vi "Check Action.vi"(6 "HRS Time":dbl, 7 "Values In":dbl[](array[numeric]), 8 "error in (no error)":errorcluster, 11 "SequencedValves in":refnum<class "TriggerDelayControl.lvclass">) -> (0 "error out":errorcluster, 2 "Actions":T1[](array[typedef]), 3 "SequencedValves out":refnum<class "TriggerDelayControl.lvclass">, 5 "Values":dbl[](array[numeric]))   [LabVIEW 2020, in "VolatusControl.lvlib" / "TriggerDelayControl.lvclass"]
uses:
  TriggerDelayControl.lvclass
  Control Action.ctl
  TriggerDelayControl.lvclass/TriggerDelayControl.ctl
  State.ctl
  Volatus/MessageQ/MessageQ.lvclass
  VolatusControl.lvlib
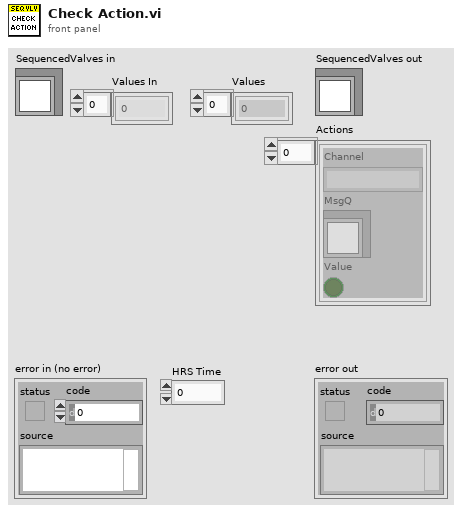
[diagram p1: front panel]
types:
  T1 = typedef "VolatusControl.lvlib/Control Action.ctl" = cluster{"Channel":string, "MsgQ":refnum<class "MessageQ.lvclass">, "Value":bool}
  T2 = typedef "VolatusControl.lvlib/TriggerDelayControl.lvclass/State.ctl" = enum16{"Idle", "Start", "Check", "Delay", "Triggered"}
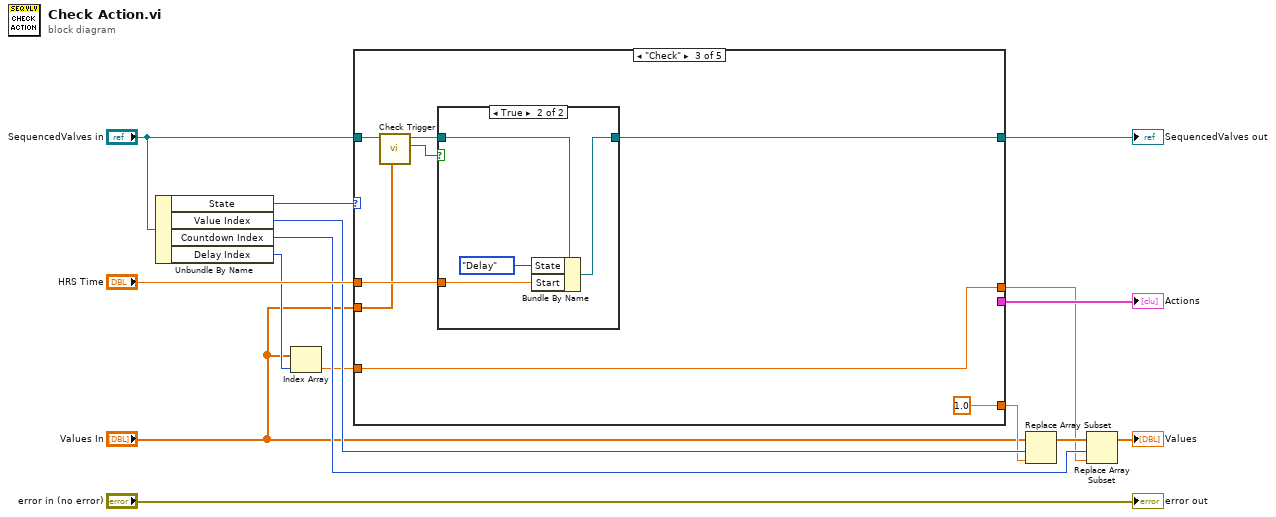
[diagram p0: block diagram]
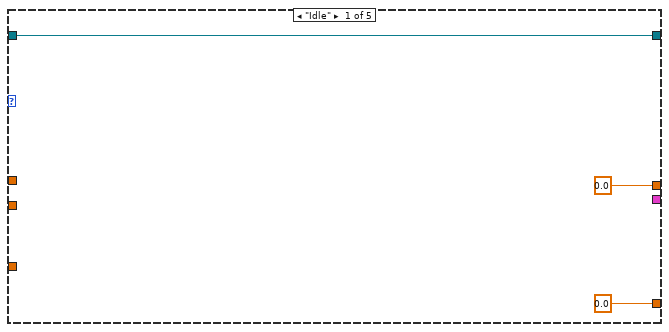
[diagram p2: hidden frame]
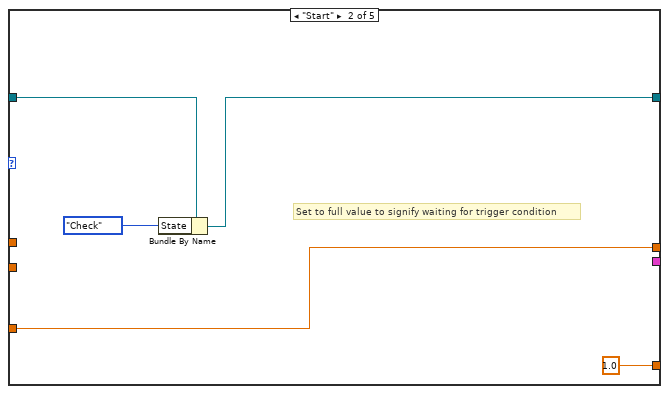
[diagram p3: hidden frame]
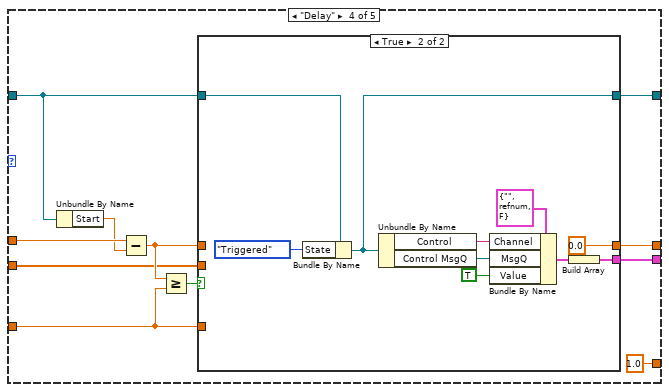
[diagram p5: hidden frame]
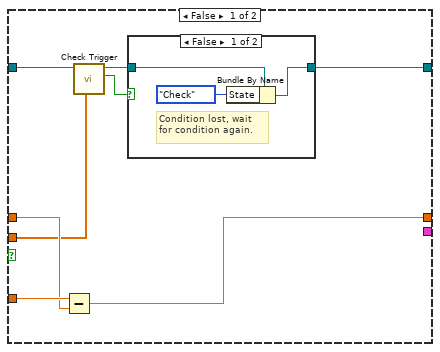
[diagram p6: hidden frame]
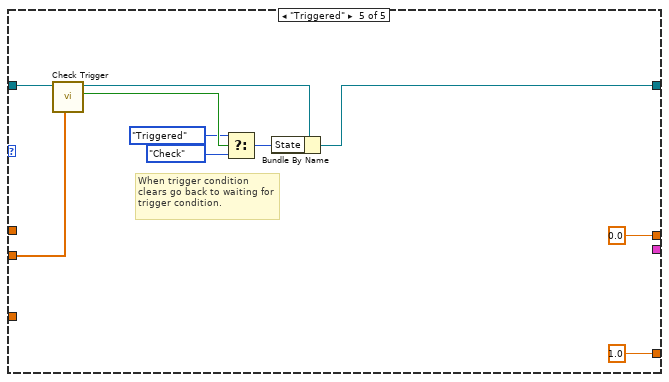
[diagram p8: hidden frame]
diagram:
  n1 = Unbundle By Name("SequencedValves in") -> ("State"=w14:T2, "Value Index"=w9:i32, "Countdown Index"=w6:i32, "Delay Index"=w4:i32)
  n2 = Index Array(array="Values In", index=w4) -> (element=w5:dbl)
  n3 = case shown="\"Check\"" w14 {
    tunnel: "SequencedValves in" -> [w18 w23 w30 w38 w78]
    tunnel: "HRS Time" -> [_ _ w29 w47 _]
    tunnel: [w18 w21 w28 w44 w73] -> w11
    tunnel: [_ _ _ w43 _] -> w10
    tunnel: [0.0 1.0 1.0 1.0 1.0] -> w8
    tunnel: w5 -> [_ w19 w31 w39 _]
    tunnel: [0.0 ("Numeric") w19 w31 w40 0.0 ("Numeric")] -> w3
    tunnel: "Values In" -> [_ _ w24 w37 w75]
    frame "Idle" {
    }
    frame "Start" {
      # "Set to full value to signify waiting for trigger condition"
      n4 = Bundle By Name(cluster=w23, "State"=State."Check") -> (w21:refnum<class "TriggerDelayControl.lvclass">)
    }
    frame "Check" {
      n5 = call "Check Trigger.vi"("Values"=w24, "TriggerDelayControl in"=w30) -> ("Triggered"=w25:bool, "TriggerDelayControl out"=w26:refnum<class "TriggerDelayControl.lvclass">)  [unwired: 7 in, 1 out]
      n6 = case shown="True" w25 {
        tunnel: w26 -> [w32 w36]
        tunnel: w29 -> [_ w34]
        tunnel: [w32 w33] -> w28
        frame False {
        }
        frame True {
          n7 = Bundle By Name(cluster=w36, "State"=State."Delay", "Start"=w34) -> (w33:refnum<class "TriggerDelayControl.lvclass">)
        }
      }
    }
    frame "Delay" {
      n8 = Unbundle By Name(w38) -> ("Start"=w46:dbl)
      n9 = Subtract(x=w47, y=w46) -> (x-y=w41:dbl)
      n10 = Greater Or Equal?(x=w41, y=w39) -> (x >= y?=w45:bool)
      n11 = case shown="True" w45 {
        tunnel: w38 -> [w52 w65]
        tunnel: [w51 w64] -> w44
        tunnel: [_ w60] -> w43
        tunnel: w41 -> [w54 _]
        tunnel: [w53 0.0] -> w40
        tunnel: w39 -> [w55 _]
        tunnel: w37 -> [w48 _]
        frame False {
          n12 = Subtract(x=w55, y=w54) -> (x-y=w53:dbl)
          n13 = call "Check Trigger.vi"("Values"=w48, "TriggerDelayControl in"=w52) -> ("Triggered"=w49:bool, "TriggerDelayControl out"=w50:refnum<class "TriggerDelayControl.lvclass">)  [unwired: 7 in, 1 out]
          n14 = case shown="False" w49 {
            tunnel: w50 -> [w58 w59]
            tunnel: [w56 w59] -> w51
            frame False {
              # "Condition lost, wait for condition again."
              n15 = Bundle By Name(cluster=w58, "State"=State."Check") -> (w56:refnum<class "TriggerDelayControl.lvclass">)
            }
            frame True {
            }
          }
        }
        frame True {
          n16 = Bundle By Name(cluster=w65, "State"=State."Triggered") -> (w64:refnum<class "TriggerDelayControl.lvclass">)
          n17 = Unbundle By Name(w64) -> ("Control"=w62:string, "Control MsgQ"=w67:refnum<class "MessageQ.lvclass">)
          n18 = Bundle By Name(cluster=T1 {"Channel"="", "MsgQ"=refnum, "Value"=FALSE} ("Action"), "Channel"=w62, "MsgQ"=w67, "Value"=TRUE) -> (w66:T1)
          n19 = Build Array(w66) -> (w60:T1[])
        }
      }
    }
    frame "Triggered" {
      # "When trigger condition clears go back to waiting for trigger condition."
      n20 = call "Check Trigger.vi"("Values"=w75, "TriggerDelayControl in"=w78) -> ("Triggered"=w74:bool, "TriggerDelayControl out"=w76:refnum<class "TriggerDelayControl.lvclass">)  [unwired: 7 in, 1 out]
      n21 = Select(t=State."Triggered" ("State"), s=w74, f=State."Check" ("State")) -> (s? t:f=w72:T2)
      n22 = Bundle By Name(cluster=w76, "State"=w72) -> (w73:refnum<class "TriggerDelayControl.lvclass">)
    }
  }
  "SequencedValves out" <- w11
  "Actions" <- w10
  n23 = Replace Array Subset(array="Values In", new element=w8, index=w9) -> (w7:dbl[])
  n24 = Replace Array Subset(array=w7, new element=w3, index=w6) -> (→"Values":dbl[])
  "error out" <- "error in (no error)"
